vi "Release.vi"   [LabVIEW 2017]
uses:
  <vilib>/FPGAPlugInAG/myRIO-1900/niLvFpga_Open_myRIO-1900.vi
  <vilib>/rvi/interface/common/dynamic/niFpgaDynamicAddResources.vi
  <vilib>/Utility/error.llb/Error Cluster From Error Code.vi
  <vilib>/rvi/errors/niLvFpgaAdjustHostInterfaceError.vi
  <vilib>/FPGAPlugInAG/Dynamic/niLvFpga_Run_Dynamic.vi
  <vilib>/FPGAPlugInAG/Dynamic/niLvFpga_Close_Dynamic.vi
  <vilib>/rvi/interface/nirviOpenFPGA/nirviOpenFPGA.xnode
  FPGA Bitfiles/BadassLoader_FPGATarget_DCMotorControlle_SJNosLHAqE0.lvbitx
  FPGA/DC Motor Controller (FPGA).vi
  <vilib>/rvi/interface/nirviReadWriteControl/nirviReadWriteControl.xnode
  <vilib>/rvi/interface/nirviMethod/nirviMethod.xnode
  <vilib>/rvi/interface/nirviCloseFPGA/nirviCloseFPGA.xnode
  NiFpgaLv.dll
  <vilib>/rvi/interface/Simulation/niFpgaSimulationCallBeginRW.vi
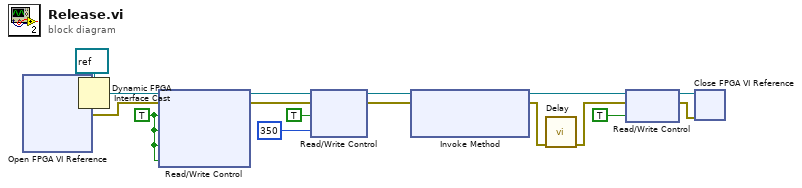
[diagram p0: block diagram]
diagram:
  w4 = TRUE ("DCmotor_0_A")
  n1 = xnode "Open FPGA VI Reference"() -> ("FPGA VI Reference Out"=w14:refnum<k20>, "error out"=w5:errorcluster)  [unwired: 2 in]
  n2 = Dynamic FPGA Interface Cast(Session In=refnum<k20> refnum ("FPGA Interface"), Type=w14) -> (Session Out=w8:refnum<k20>)
  n3 = xnode "Read/Write Control"("FPGA VI Reference In"=w8, "error in"=w5, "DCmotor_0_A"=w4, "DCmotor_0_B"=w4, "DCmotor_1_A"=w4, "DCmotor_1_B"=w4) -> ("FPGA VI Reference Out"=w7:refnum<k20>, "error out"=w6:errorcluster)
  n4 = xnode "Read/Write Control"("FPGA VI Reference In"=w7, "error in"=w6, "S 6"=TRUE, "Servo 6"=u32 350) -> ("FPGA VI Reference Out"=w12:refnum<k20>, "error out"=w11:errorcluster)
  n5 = xnode "Invoke Method"("FPGA VI Reference In"=w12, "error in"=w11) -> ("FPGA VI Reference Out"=w2:refnum<k20>, "error out"=w9:errorcluster)  [unwired: 1 in]
  n6 = call "Delay"("error in (no error)"=w9) -> ("error out"=w1:errorcluster)  [unwired: 10 in]
  n7 = xnode "Read/Write Control"("FPGA VI Reference In"=w2, "error in"=w1, "stop"=TRUE) -> ("FPGA VI Reference Out"=w17:refnum<k20>, "error out"=w16:errorcluster)
  n8 = xnode "Close FPGA VI Reference"("FPGA VI Reference In"=w17, "error in"=w16) -> ()  [unwired: 1 out]
